vi "cansub_rp1210_xnet_lv2021.vi"() -> ()   [LabVIEW 2021]
uses:
  <vilib>/xnet/xnet.llb/XNET Create Session (Generic).vi
  <vilib>/xnet/xnet.llb/XNET Mode.ctl
  <vilib>/xnet/xnet.llb/XNET Convert (Frame Raw to Signal).vi
  <vilib>/xnet/xnet.llb/XNET Convert (Signal to Frame Raw).vi
panel:
  in  "Send period (s)":dbl=0.1 caption="Time Target (s)"
  in  "Send":bool
  out "Frames sent":i32
  in  "Send values":dbl[](array[numeric])=[1500.0, 1.0] caption="signal data" format="%.2f"
  in  "Send signals":string[](array[string])=["RigCommand.TargetSpeed", "RigCommand.Enable"]
  out "Chart":dbl(graph)=5262.25
  in  "Chart signal #":i32
  in  "stop":bool
  out "Signal values":dbl[](array[numeric]) caption="signal data" format="%.2f"
  out "Frames read":i32
  out "Bytes read":i32
  out "Client ID":i16
  in  "Protocol":string="CAN:Baud=500"
  in  "Device ID":i16=1
  in  "DBC file (empty: labview-demo.dbc beside this VI)":string
  in  "Signals":string[](array[string])=["EngineData.EngineSpeed", "EngineData.EngineTorque", "EngineData.CoolantTemp", "VehicleData.VehicleSpeed", "VehicleData.BatteryVoltage"]
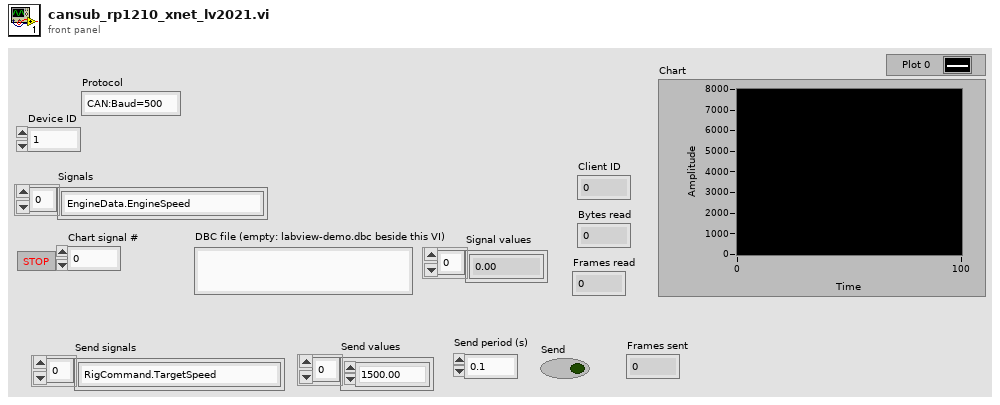
[diagram p1: front panel]
types:
  T1 = typedef "XNET Mode.ctl" = u32
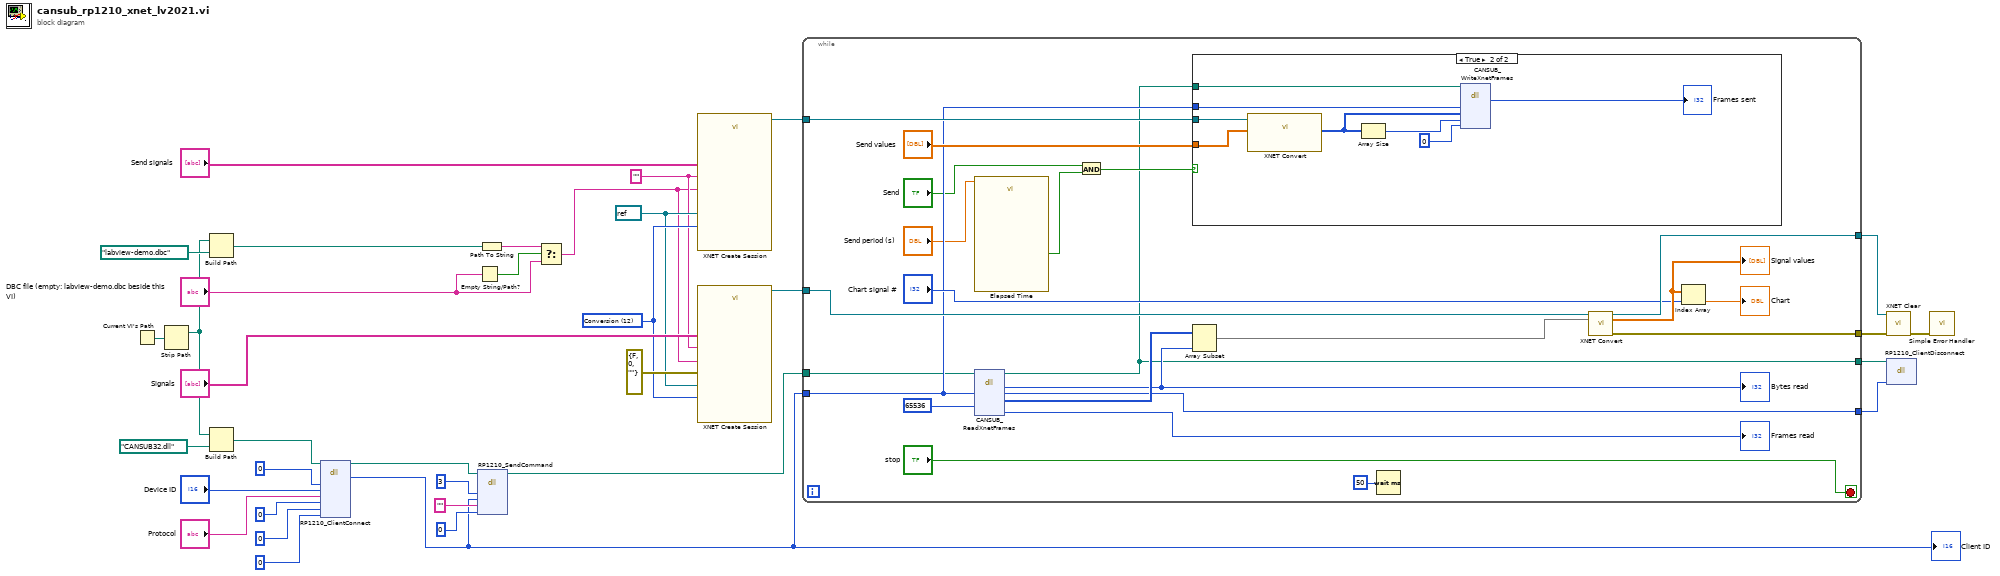
[diagram p0: block diagram]
diagram:
  w16 = "" ("cluster (empty)")
  w17 = refnum<k21> refnum ("interface")
  w18 = T1 12 items=["Signal Input Single-point", "Signal Input Waveform", "Signal Input XY", "Signal Output Single-point", "Signal Output Waveform", "Signal Output XY", "Frame Input Stream", "Frame Input Queued", "Frame Input Single-point", "Frame Output Stream", "Frame Output Queued", "Frame Output Single-point", "Conversion"] ("mode")
  n1 = Current VI's Path() -> (path=w14:path)
  n2 = Strip Path(path=w14) -> (stripped path=w6:path)  [unwired: 1 out]
  n3 = Build Path(base path=w6, name or relative path=path "labview-demo.dbc") -> (appended path=w13:path)
  n4 = Build Path(base path=w6, name or relative path=path "CANSUB32.dll") -> (appended path=w4:path)
  n5 = dll-call lib="CANSUB32.dll" fn="RP1210_ClientConnect"(path in=w4, "hwnd"=i64 0, "device"="Device ID", "protocol"="Protocol", "tx"=0, "rx"=0, "appPacketizing"=i16 0) -> (path out=w3:path, "return type"=w24:i16)  [unwired: 8 in, 1 out]
  "Client ID" <- w24
  n6 = Empty String/Path?(string/path="DBC file (empty: labview-demo.dbc beside this VI)") -> (empty?=w11:bool)
  n7 = dll-call lib="CANSUB32.dll" fn="RP1210_SendCommand" label="RP1210_SendCommand (3 = all filters pass)"(path in=w3, "command"=i16 3, "client"=w24, "data"="", "size"=i16 0) -> (path out=w2:path)  [unwired: 7 in, 1 out]
  n8 = Path To String(path=w13) -> (string=w10:string)
  n9 = Select(t=w10, s=w11, f="DBC file (empty: labview-demo.dbc beside this VI)") -> (s? t:f=w8:string)
  n10 = call-poly <vilib>:"XNET Create Session.vi"("list (empty)"="Send signals", "mode"=w18, "interface"=w17, "database (:memory:)"=w8, "cluster (empty)"=w16) -> ("session out"=w7:refnum<k21>)  [unwired: 9 in, 1 out]
  n11 = call-poly <vilib>:"XNET Create Session.vi"("list (empty)"="Signals", "mode"=w18, "interface"=w17, "error in (no error)"=errorcluster {"status"=FALSE, "code"=0, "source"=""}, "database (:memory:)"=w8, "cluster (empty)"=w16) -> ("session out"=w25:refnum<k21>)  [unwired: 8 in, 1 out]
  n12 = while {
    tunnel: w25 -> [w53]
    tunnel: w24 -> [w42]
    tunnel: [w50] -> w23
    tunnel: [w49] -> w22
    tunnel: [w48] -> w21
    tunnel: w7 -> [w43]
    tunnel: w2 -> [w37]
    tunnel: [w36] -> w1
    stop <- "stop" stop-if-true
    n13 = call "Elapsed Time"("Time Target (s)"="Send period (s)") -> ("Time has Elapsed"=w41:bool)  [unwired: 11 in, 7 out]
    n14 = dll-call lib="CANSUB32.dll" fn="CANSUB_ReadXnetFrames"(path in=w37, "client"=w42, "size"=65536) -> (path out=w36:path, "return type"=w55:i32, "client"=w50:i16, "buffer"=w56:u8[], "count"=→"Frames read":i32)  [unwired: 5 in, 1 out]
    "Bytes read" <- w55
    n15 = And(x="Send", y=w41) -> (x .and. y?=w40:bool)
    n16 = case shown="True" w40 {
      tunnel: "Send values" -> [_ w66]
      tunnel: w43 -> [_ w65]
      tunnel: w42 -> [_ w62]
      tunnel: w36 -> [_ w59]
      frame False {
      }
      frame True {
        n17 = call-poly <vilib>:"XNET Convert.vi"("session in"=w65, "signal data"=w66) -> ("frame data"=w64:u8[])  [unwired: 11 in, 2 out]
        n18 = Array Size(array=w64) -> (size(s)=w63:i32)
        n19 = dll-call lib="CANSUB32.dll" fn="CANSUB_WriteXnetFrames"(path in=w59, "client"=w62, "buffer"=w64, "size"=w63, "count"=0) -> ("return type"=→"Frames sent":i32)  [unwired: 6 in, 2 out]
      }
    }
    n20 = Array Subset(array=w56, length=w55) -> (w54:u8[])  [unwired: 1 in]
    n21 = Wait (ms)(milliseconds to wait=u32 50) -> ()  [unwired: 1 out]
    n22 = call-poly <vilib>:"XNET Convert.vi"("session in"=w53, "frame data"=w54) -> ("session out"=w49:refnum<k21>, "signal data"=w47:dbl[], "error out"=w48:errorcluster)  [unwired: 11 in]
    "Signal values" <- w47
    n23 = Index Array(array=w47, index="Chart signal #") -> (element=→"Chart":dbl)
  }
  n24 = call <vilib>:"XNET Clear.vi"("session in"=w22, "error in (no error)"=w21) -> ("error out"=w20:errorcluster)  [unwired: 13 in]
  n25 = dll-call lib="CANSUB32.dll" fn="RP1210_ClientDisconnect"(path in=w1, "client"=w23) -> ()  [unwired: 4 in, 2 out]
  n26 = call <vilib>:"Simple Error Handler.vi"("error in (no error)"=w20) -> ()  [unwired: 4 in, 5 out]
